vi "DAC Configure.vi"(8 "error in":errorcluster, 11 "DAC CS Humid in":refnum<class "DAC CS Humid.lvclass">) -> (0 "error out":errorcluster, 3 "DAC CS Humid out":refnum<class "DAC CS Humid.lvclass">)   [LabVIEW 2019, in "DAC.lvlib" / "DAC CS Humid.lvclass"]
uses:
  DAC CS Humid.lvclass
  C:/Users/krio/Documents/LV_Projects/test-stand/App/DAC/DAC.lvclass
  DAC.lvclass/DAC.ctl
  DAC CS Humid.lvclass/DAC CS Humid.ctl
  <vilib>/DAQmx/create/scale.llb/DAQmx Create Scale (Map Ranges).vi
  <vilib>/DAQmx/create/channels.llb/DAQmx Create Channel (AI-Current-Basic).vi
  DAC.lvclass
  <resource>/objmgr/daqmx.rc
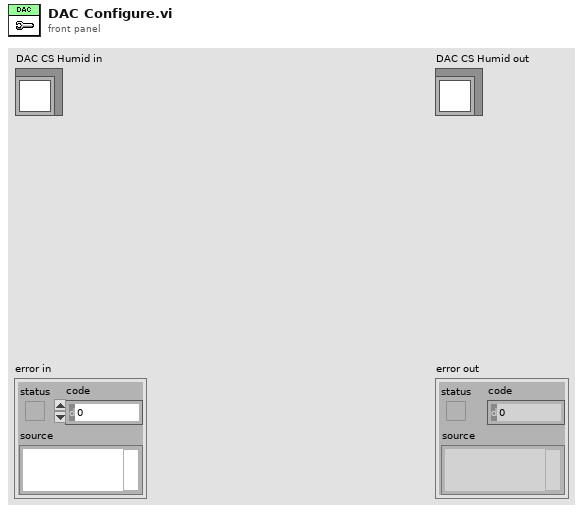
[diagram p1: front panel]
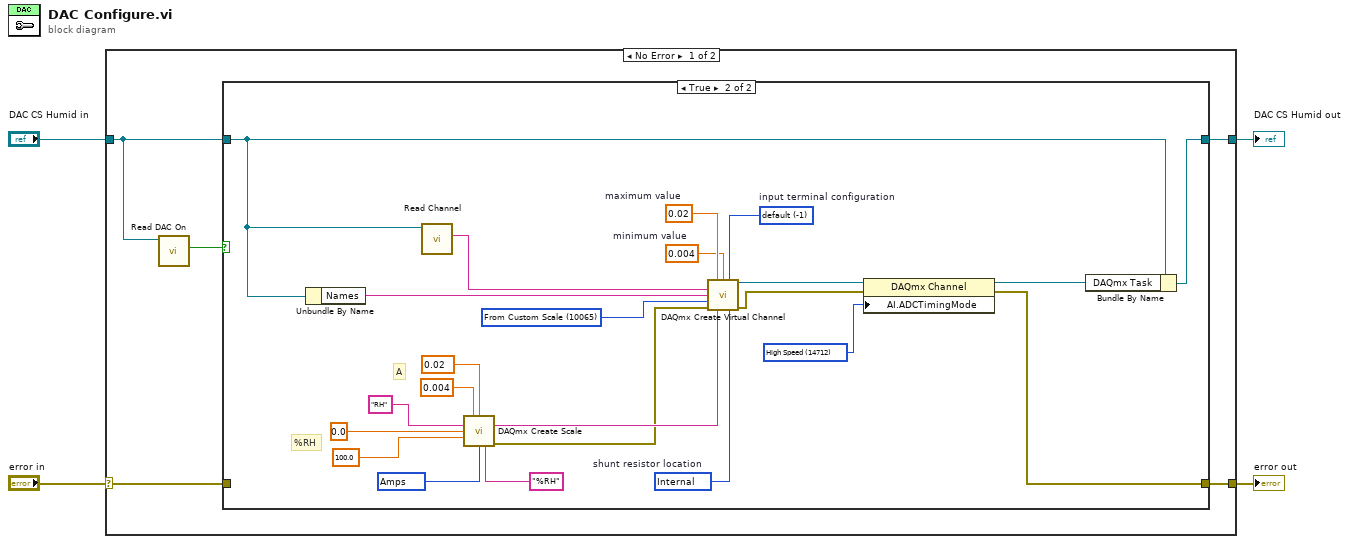
[diagram p0: block diagram]
diagram:
  n1 = case shown="No Error" "error in" {
    selector: "error in" -> [w6 w36]
    tunnel: [w5 w36] -> w4
    tunnel: [w7 w35] -> w3
    tunnel: "DAC CS Humid in" -> [w9 w35]
    frame No Error {
      n2 = call "Read DAC On.vi"("DAC in"=w9) -> ("DAC On"=w8:bool)  [unwired: 8 in, 2 out]
      n3 = case shown="True" w8 {
        tunnel: w9 -> [w11 w32]
        tunnel: [w11 w34] -> w7
        tunnel: w6 -> [w10 _]
        tunnel: [w10 w12] -> w5
        frame False {
        }
        frame True {
          w13 = 14712 items=["Automatic"=16097, "High Resolution"=10195, "High Speed"=14712, "Best 50 Hz Rejection"=14713, "Best 60 Hz Rejection"=14714, "Custom"=10137] ("AI.ADCTimingMode")
          w18 = 10342 items=["Volts"=10348, "Amps"=10342, "Deg F"=10144, "Deg C"=10143, "Deg R"=10145, "Kelvins"=10325, "Strain"=10299, "Ohms"=10384, "Hz"=10373, "Seconds"=10364, "Meters"=10219, "Inches"=10379, "Degrees"=10146, "Radians"=10273, "Ticks"=10304, "g"=10186, "m/s^2"=12470, "m/s"=15959, "in/s"=15960, "Pascals"=10081, "Newtons"=15875, "Pounds"=15876, "kgf"=15877, "psi"=15879, "bar"=15880, "Nm"=15881, "oz-in"=15882, "lb-in"=15883, "lb-ft"=15884, "Volts/Volt"=15896, "mVolts/Volt"=15897, "pCoulombs"=16103, "Coulombs"=16102, "From TEDS"=12516] ("pre-scaled units")
          w26 = 10200 items=["default"=-1, "Internal"=10200, "External"=10167]  # shunt resistor location
          w27 = -1 items=["default"=-1, "RSE"=10083, "NRSE"=10078, "Differential"=10106, "Pseudodifferential"=12529]  # input terminal configuration
          w28 = 10065 items=["Amps"=10342, "From Custom Scale"=10065] ("units")
          w29 = 0.004  # minimum value
          w30 = 0.02  # maximum value
          # "%RH"
          # "A"
          n4 = Unbundle By Name(w32) -> ("Names"=w33:string)
          n5 = call "Read Channel.vi"("DAC in"=w32) -> ("Channel"=w31:string)  [unwired: 8 in, 2 out]
          n6 = call-poly <vilib>:"DAQmx Create Scale.vi"("pre-scaled minimum"=0.004, "pre-scaled maximum"=0.02, "name"="RH", "scaled minimum"=0.0, "scaled maximum"=100.0, "pre-scaled units"=w18, "scaled units"="%RH") -> ("scale out"=w25:tag, "error out"=w19:errorcluster)  [unwired: 7 in]
          n7 = call-poly <vilib>:"DAQmx Create Virtual Channel.vi"("maximum value"=w30, "minimum value"=w29, "input terminal configuration"=w27, "physical channels"=w31, "name to assign"=w33, "units"=w28, "error in"=w19, "custom scale name"=w25, "shunt resistor location"=w26) -> ("task out"=w16:refnum<k21>, "error out"=w14:errorcluster)  [unwired: 5 in]
          n8 = property class="DAQmx Channel"(reference=w16, error in=w14, "AI.ADCTimingMode"=w13) -> (reference out=w15:refnum<k21>, error out=w12:errorcluster)
          n9 = Bundle By Name(cluster=w32, "DAQmx Task"=w15) -> (w34:refnum<class "DAC CS Humid.lvclass">)
        }
      }
    }
    frame Error {
    }
  }
  "error out" <- w4
  "DAC CS Humid out" <- w3
